vi "RemoteVI Target Running.vi"(0 "VI":refnum<vi>, 5 "window":u64) -> (4 "running?":bool)   [LabVIEW 2020, in "RemoteVI.lvlib"]
doc: "Whether what is shared still runs: window 0 - VI's Execution:State is Run Top Level or Running (2 or more); a window target - the window still exists (user32 IsWindow.vi, no VI Server call). An error reading the state counts as not running."
uses:
  RemoteVI.lvlib
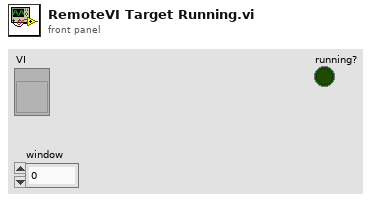
[diagram p1: front panel]
types:
  T1 = enum32{"Bad", "Idle", "Run top level", "Running"}
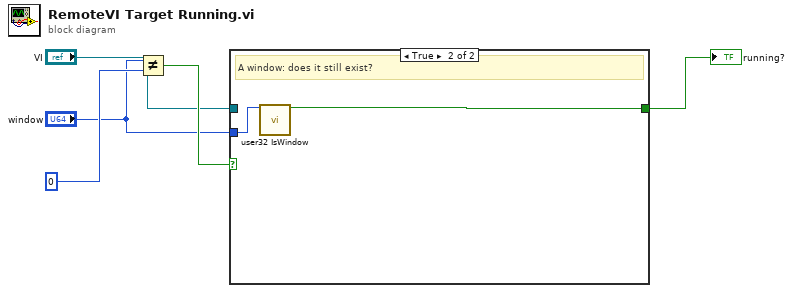
[diagram p0: block diagram]
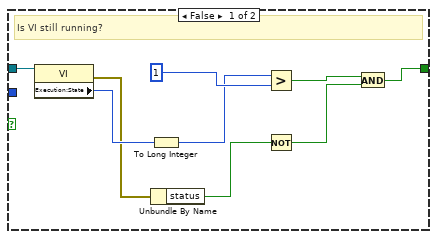
[diagram p2: hidden frame]
diagram:
  n1 = Not Equal?(x="window", y=u64 0) -> (x != y?=w4:bool)
  n2 = case shown="True" w4 {
    tunnel: "VI" -> [w6 _]
    tunnel: "window" -> [_ w15]
    tunnel: [w14 w16] -> w5
    frame False {
      # "Is VI still running?"
      n3 = property class="VI"(reference=w6) -> (error out=w7:errorcluster, "Execution:State"=w8:T1)  [unwired: 1 in, 1 out]
      n4 = To Long Integer(number=w8) -> (32bit integer=w9:i32)
      n5 = Unbundle By Name(w7) -> ("status"=w12:bool)
      n6 = Greater?(x=w9, y=1) -> (0:w11:bool)
      n7 = Not(x=w12) -> (.not. x?=w13:bool)
      n8 = And(x=w11, y=w13) -> (x .and. y?=w14:bool)
    }
    frame True {
      # "A window: does it still exist?"
      n9 = call "user32 IsWindow.vi"("hWnd"=w15) -> ("window?"=w16:bool)  [unwired: 13 in, 1 out]
    }
  }
  "running?" <- w5
